vi "CC_T2_Manipulation.vi"(8 "Invert?":bool, 9 "Tau Step Size":dbl=2e-09, 10 "Numeric 2":i32, 11 "Numeric":i32) -> (2 "Tau":dbl)   [LabVIEW 2024]
uses:
  <vilib>/Utility/error.llb/DialogTypeEnum.ctl
  SpinCore_API_file_location.vi
panel:
  in  "# of Instructions":u32=33
  in  "Instructions":T1(array[cluster])=[{"Instruct Data"=0, "Op Code"=0, "Flags"=[FALSE, FALSE, TRUE, FALSE, FALSE, FALSE, FALSE, TRUE, FALSE, FALSE, FALSE, FALSE, FALSE, FALSE, FALSE, FALSE, FALSE, FALSE, FALSE, FALSE, FALSE, FALSE, FALSE, TRUE], "Comments"="0 Triggers", "Time (s)"=1e-07}, {"Instruct Data"=0, "Op Code"=0, "Flags"=[FALSE, FALSE, FALSE, FALSE, FALSE, FALSE, FALSE, TRUE, FALSE, FALSE, FALSE, FALSE, FALSE, FALSE, FALSE, FALSE, FALSE, FALSE, FALSE, FALSE, FALSE, FALSE, FALSE, FALSE], "Comments"="1 Dark ", "Time (s)"=5e-05}, {"Instruct Data"=0, "Op Code"=0, "Flags"=[FALSE, FALSE, FALSE, FALSE, FALSE, FALSE, FALSE, TRUE, FALSE, FALSE, FALSE, FALSE, FALSE, FALSE, FALSE, FALSE, FALSE, FALSE, FALSE, FALSE, FALSE, FALSE, FALSE, FALSE], "Comments"="2 AOM Buffer", "Time (s)"=5e-07}, {"Instruct Data"=0, "Op Code"=0, "Flags"=[TRUE, FALSE, FALSE, TRUE, FALSE, FALSE, FALSE, TRUE, FALSE, FALSE, FALSE, FALSE, FALSE, FALSE, FALSE, FALSE, FALSE, FALSE, FALSE, FALSE, FALSE, FALSE, FALSE, FALSE], "Comments"="3 pi/2_X", "Time (s)"=3.6e-08}, {"Instruct Data"=0, "Op Code"=0, "Flags"=[FALSE, FALSE, FALSE, FALSE, FALSE, FALSE, FALSE, TRUE, FALSE, FALSE, FALSE, FALSE, FALSE, FALSE, FALSE, FALSE, FALSE, FALSE, FALSE, FALSE, FALSE, FALSE, FALSE, FALSE], "Comments"="4 tau", "Time (s)"=2.1e-06}, {"Instruct Data"=0, "Op Code"=0, "Flags"=[TRUE, FALSE, FALSE, TRUE, FALSE, FALSE, FALSE, TRUE, FALSE, FALSE, FALSE, FALSE, FALSE, FALSE, FALSE, FALSE, FALSE, FALSE, FALSE, FALSE, FALSE, FALSE, FALSE, FALSE], "Comments"="5  Pi_X", "Time (s)"=6.7e-08}, {"Instruct Data"=0, "Op Code"=0, "Flags"=[FALSE, FALSE, FALSE, FALSE, FALSE, FALSE, FALSE, TRUE, FALSE, FALSE, FALSE, FALSE, FALSE, FALSE, FALSE, FALSE, FALSE, FALSE, FALSE, FALSE, FALSE, FALSE, FALSE, FALSE], "Comments"="6 Tau", "Time (s)"=2.1e-06}, {"Instruct Data"=0, "Op Code"=0, "Flags"=[TRUE, FALSE, FALSE, FALSE, TRUE, FALSE, FALSE, TRUE, FALSE, FALSE, FALSE, FALSE, FALSE, FALSE, FALSE, FALSE, FALSE, FALSE, FALSE, FALSE, FALSE, FALSE, FALSE, FALSE], "Comments"="7 Pi/2_Y", "Time (s)"=3.9e-08}, {"Instruct Data"=0, "Op Code"=0, "Flags"=[FALSE, FALSE, FALSE, FALSE, FALSE, FALSE, FALSE, TRUE, FALSE, FALSE, FALSE, FALSE, FALSE, FALSE, FALSE, FALSE, FALSE, FALSE, FALSE, FALSE, FALSE, FALSE, FALSE, FALSE], "Comments"="8 Tau CC", "Time (s)"=1e-08}, {"Instruct Data"=0, "Op Code"=0, "Flags"=[TRUE, FALSE, FALSE, TRUE, FALSE, FALSE, FALSE, TRUE, FALSE, FALSE, FALSE, FALSE, FALSE, FALSE, FALSE, FALSE, FALSE, FALSE, FALSE, FALSE, FALSE, FALSE, FALSE, FALSE], "Comments"="9 pi/2_X", "Time (s)"=3.6e-08}, {"Instruct Data"=0, "Op Code"=0, "Flags"=[FALSE, FALSE, FALSE, FALSE, FALSE, FALSE, FALSE, TRUE, FALSE, FALSE, FALSE, FALSE, FALSE, FALSE, FALSE, FALSE, FALSE, FALSE, FALSE, FALSE, FALSE, FALSE, FALSE, FALSE], "Comments"="10 tau", "Time (s)"=2.1e-06}, {"Instruct Data"=0, "Op Code"=0, "Flags"=[TRUE, FALSE, FALSE, TRUE, FALSE, FALSE, FALSE, TRUE, FALSE, FALSE, FALSE, FALSE, FALSE, FALSE, FALSE, FALSE, FALSE, FALSE, FALSE, FALSE, FALSE, FALSE, FALSE, FALSE], "Comments"="11  Pi_X", "Time (s)"=6.7e-08}, {"Instruct Data"=0, "Op Code"=0, "Flags"=[FALSE, FALSE, FALSE, FALSE, FALSE, FALSE, FALSE, TRUE, FALSE, FALSE, FALSE, FALSE, FALSE, FALSE, FALSE, FALSE, FALSE, FALSE, FALSE, FALSE, FALSE, FALSE, FALSE, FALSE], "Comments"="12 tau", "Time (s)"=2.1e-06}, {"Instruct Data"=0, "Op Code"=0, "Flags"=[TRUE, FALSE, FALSE, FALSE, TRUE, FALSE, FALSE, TRUE, FALSE, FALSE, FALSE, FALSE, FALSE, FALSE, FALSE, FALSE, FALSE, FALSE, FALSE, FALSE, FALSE, FALSE, FALSE, FALSE], "Comments"="13 pi/2_Y", "Time (s)"=3.7e-08}, {"Instruct Data"=0, "Op Code"=0, "Flags"=[FALSE, TRUE, FALSE, FALSE, FALSE, FALSE, FALSE, TRUE, FALSE, FALSE, FALSE, FALSE, FALSE, FALSE, FALSE, FALSE, FALSE, FALSE, FALSE, FALSE, FALSE, FALSE, FALSE, FALSE], "Comments"="14 AOM Delay", "Time (s)"=5e-07}, {"Instruct Data"=0, "Op Code"=0, "Flags"=[FALSE, TRUE, FALSE, FALSE, FALSE, FALSE, FALSE, FALSE, FALSE, FALSE, FALSE, FALSE, FALSE, FALSE, FALSE, FALSE, FALSE, FALSE, FALSE, FALSE, FALSE, FALSE, FALSE, FALSE], "Comments"="15 inhibit off", "Time (s)"=5e-07}, {"Instruct Data"=0, "Op Code"=0, "Flags"=[FALSE, TRUE, FALSE, FALSE, FALSE, FALSE, FALSE, TRUE, FALSE, FALSE, FALSE, FALSE, FALSE, FALSE, FALSE, FALSE, FALSE, FALSE, FALSE, FALSE, FALSE, FALSE, FALSE, FALSE], "Comments"="16 AOM", "Time (s)"=5e-06}, {"Instruct Data"=0, "Op Code"=0, "Flags"=[FALSE, FALSE, FALSE, FALSE, FALSE, FALSE, FALSE, TRUE, FALSE, FALSE, FALSE, FALSE, FALSE, FALSE, FALSE, FALSE, FALSE, FALSE, FALSE, FALSE, FALSE, FALSE, FALSE, FALSE], "Comments"="17 Dark", "Time (s)"=5e-05}, {"Instruct Data"=0, "Op Code"=0, "Flags"=[FALSE, FALSE, FALSE, FALSE, FALSE, FALSE, FALSE, TRUE, FALSE, FALSE, FALSE, FALSE, FALSE, FALSE, FALSE, FALSE, FALSE, FALSE, FALSE, FALSE, FALSE, FALSE, FALSE, FALSE], "Comments"="18 AOM Delay", "Time (s)"=5e-07}, {"Instruct Data"=0, "Op Code"=0, "Flags"=[TRUE, FALSE, FALSE, TRUE, FALSE, FALSE, FALSE, TRUE, FALSE, FALSE, FALSE, FALSE, FALSE, FALSE, FALSE, FALSE, FALSE, FALSE, FALSE, FALSE, FALSE, FALSE, FALSE, FALSE], "Comments"="19 pi/2_X ", "Time (s)"=3.6e-08}, {"Instruct Data"=0, "Op Code"=0, "Flags"=[FALSE, FALSE, FALSE, FALSE, FALSE, FALSE, FALSE, TRUE, FALSE, FALSE, FALSE, FALSE, FALSE, FALSE, FALSE, FALSE, FALSE, FALSE, FALSE, FALSE, FALSE, FALSE, FALSE, FALSE], "Comments"="20 tau", "Time (s)"=2.1e-06}, {"Instruct Data"=0, "Op Code"=0, "Flags"=[TRUE, FALSE, FALSE, TRUE, FALSE, FALSE, FALSE, TRUE, FALSE, FALSE, FALSE, FALSE, FALSE, FALSE, FALSE, FALSE, FALSE, FALSE, FALSE, FALSE, FALSE, FALSE, FALSE, FALSE], "Comments"="21 Pi_x", "Time (s)"=6.7e-08}, {"Instruct Data"=0, "Op Code"=0, "Flags"=[FALSE, FALSE, FALSE, FALSE, FALSE, FALSE, FALSE, TRUE, FALSE, FALSE, FALSE, FALSE, FALSE, FALSE, FALSE, FALSE, FALSE, FALSE, FALSE, FALSE, FALSE, FALSE, FALSE, FALSE], "Comments"="22 tau", "Time (s)"=2.1e-06}, {"Instruct Data"=0, "Op Code"=0, "Flags"=[TRUE, FALSE, FALSE, FALSE, TRUE, FALSE, FALSE, TRUE, FALSE, FALSE, FALSE, FALSE, FALSE, FALSE, FALSE, FALSE, FALSE, FALSE, FALSE, FALSE, FALSE, FALSE, FALSE, FALSE], "Comments"="23 pi/2 _Y", "Time (s)"=3.9e-08}, {"Instruct Data"=0, "Op Code"=0, "Flags"=[FALSE, FALSE, FALSE, FALSE, FALSE, FALSE, FALSE, TRUE, FALSE, FALSE, FALSE, FALSE, FALSE, FALSE, FALSE, FALSE, FALSE, FALSE, FALSE, FALSE, FALSE, FALSE, FALSE, FALSE], "Comments"="24 Tau_CC", "Time (s)"=1e-08}, {"Instruct Data"=0, "Op Code"=0, "Flags"=[TRUE, FALSE, FALSE, TRUE, FALSE, FALSE, FALSE, TRUE, FALSE, FALSE, FALSE, FALSE, FALSE, FALSE, FALSE, FALSE, FALSE, FALSE, FALSE, FALSE, FALSE, FALSE, FALSE, FALSE], "Comments"="25 pi/2_X", "Time (s)"=3.6e-08}, {"Instruct Data"=0, "Op Code"=0, "Flags"=[FALSE, FALSE, FALSE, FALSE, FALSE, FALSE, FALSE, TRUE, FALSE, FALSE, FALSE, FALSE, FALSE, FALSE, FALSE, FALSE, FALSE, FALSE, FALSE, FALSE, FALSE, FALSE, FALSE, FALSE], "Comments"="26 tau", "Time (s)"=2.1e-06}, {"Instruct Data"=0, "Op Code"=0, "Flags"=[TRUE, FALSE, FALSE, TRUE, FALSE, FALSE, FALSE, TRUE, FALSE, FALSE, FALSE, FALSE, FALSE, FALSE, FALSE, FALSE, FALSE, FALSE, FALSE, FALSE, FALSE, FALSE, FALSE, FALSE], "Comments"="27 Pi_X", "Time (s)"=6.7e-08}, {"Instruct Data"=0, "Op Code"=0, "Flags"=[FALSE, FALSE, FALSE, FALSE, FALSE, FALSE, FALSE, TRUE, FALSE, FALSE, FALSE, FALSE, FALSE, FALSE, FALSE, FALSE, FALSE, FALSE, FALSE, FALSE, FALSE, FALSE, FALSE, FALSE], "Comments"="28 tau", "Time (s)"=2.1e-06}, {"Instruct Data"=0, "Op Code"=0, "Flags"=[TRUE, FALSE, FALSE, FALSE, TRUE, FALSE, FALSE, TRUE, FALSE, FALSE, FALSE, FALSE, FALSE, FALSE, FALSE, FALSE, FALSE, FALSE, FALSE, FALSE, FALSE, FALSE, FALSE, FALSE], "Comments"="29 3pi/2_Y", "Time (s)"=1.05e-07}, {"Instruct Data"=0, "Op Code"=0, "Flags"=[FALSE, TRUE, FALSE, FALSE, FALSE, FALSE, FALSE, TRUE, FALSE, FALSE, FALSE, FALSE, FALSE, FALSE, FALSE, FALSE, FALSE, FALSE, FALSE, FALSE, FALSE, FALSE, FALSE, FALSE], "Comments"="30  aom delay", "Time (s)"=5e-07}, {"Instruct Data"=0, "Op Code"=0, "Flags"=[FALSE, TRUE, FALSE, FALSE, FALSE, FALSE, FALSE, FALSE, FALSE, FALSE, FALSE, FALSE, FALSE, FALSE, FALSE, FALSE, FALSE, FALSE, FALSE, FALSE, FALSE, FALSE, FALSE, FALSE], "Comments"="31inhibit off", "Time (s)"=5e-07}, {"Instruct Data"=0, "Op Code"=6, "Flags"=[FALSE, TRUE, FALSE, FALSE, FALSE, FALSE, FALSE, TRUE, FALSE, FALSE, FALSE, FALSE, FALSE, FALSE, FALSE, FALSE, FALSE, FALSE, FALSE, FALSE, FALSE, FALSE, FALSE, FALSE], "Comments"="32  aom", "Time (s)"=5e-06}, {"Instruct Data"=0, "Op Code"=0, "Flags"=[TRUE, FALSE, FALSE, TRUE, FALSE, FALSE, FALSE, TRUE, FALSE, FALSE, FALSE, FALSE, FALSE, FALSE, FALSE, FALSE, FALSE, FALSE, FALSE, FALSE, FALSE, FALSE, FALSE, FALSE], "Comments"="33 AOM", "Time (s)"=9.2e-08}] {"Time (s)" format="%.3p"; "Op Code" items=["Continue", "Stop", "Loop", "End Loop", "JSR", "RTS", "Branch", "Long Delay", "Wait"]}
  out "output array":T1(array[cluster])
  in  "clock_freq (MHz)":dbl=500.0
  out "x+y 2":dbl
  out "x+y 5":dbl
  out "x+y 6":dbl
  out "output array 2":T1(array[cluster])
  in  "clock_freq (MHz) 2":dbl=500.0
  out "x+y 11":dbl
  out "x+y 8":dbl
  out "x+y 7":dbl
  # "1) MW indication\n2)AOM\n3) SR400 trigger\n4) I\n5) Q\n8) inhibit\n24) oss trigger"
  # "1"
  # "2"
  # "3"
  # "4"
  # "5"
  # "6"
  # "7"
  # "8"
  # "9"
  # "10"
  # "11"
  # "12"
  # "13"
  # "14"
  # "15"
  # "16"
  # "17"
  # "18"
  # "19"
  # "20"
  # "21"
  # "22"
  # "23"
  # "24"
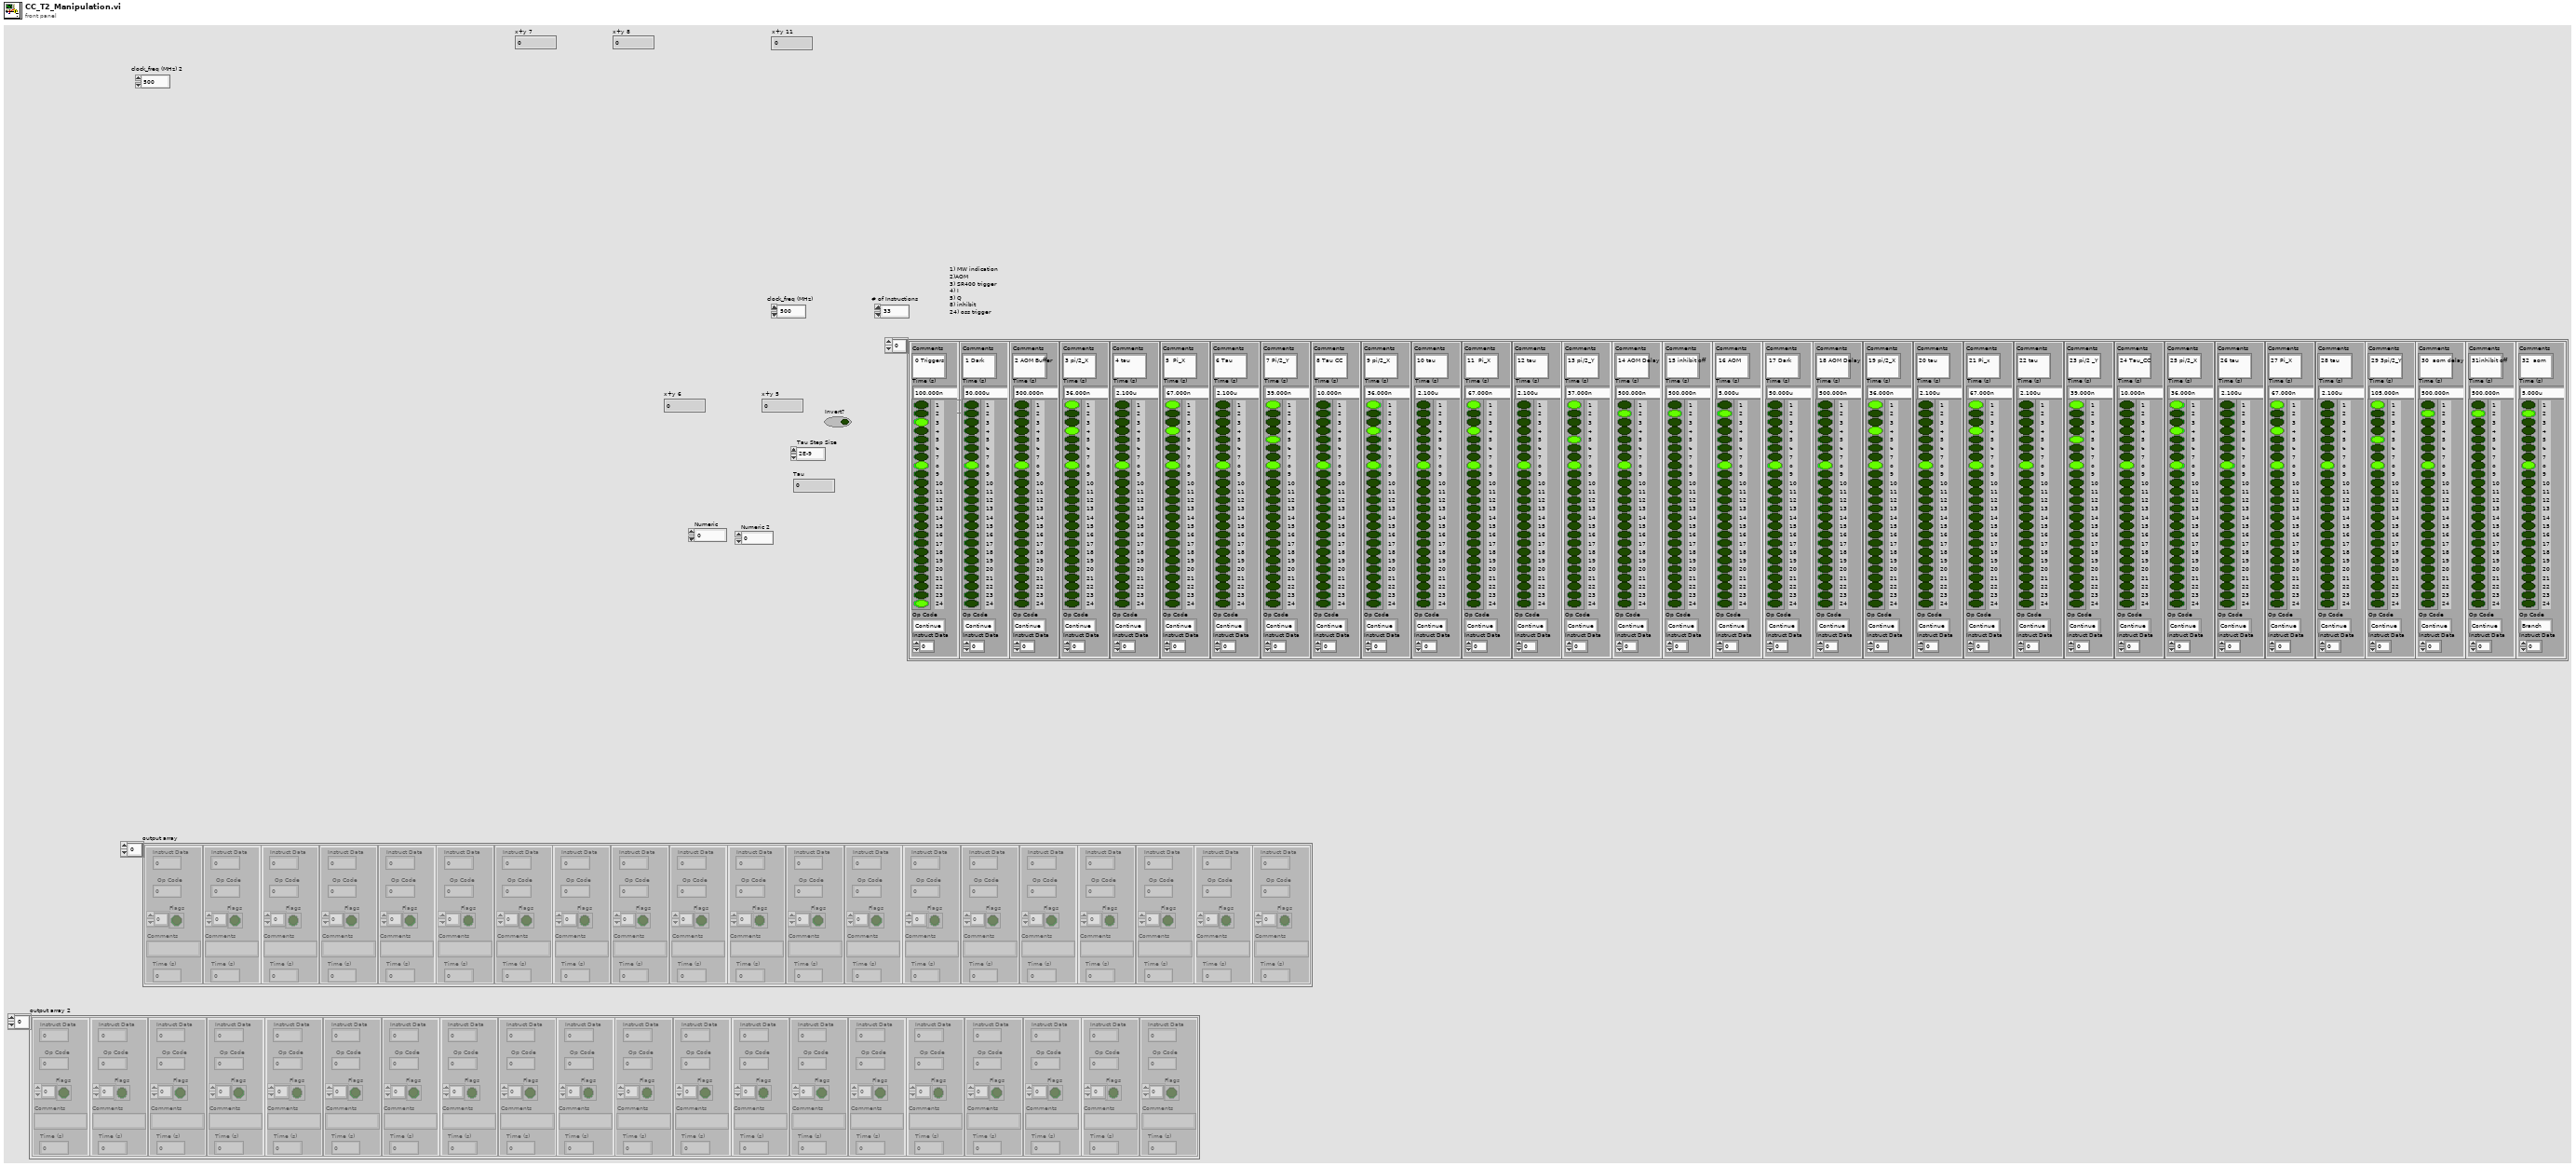
[diagram p1: front panel]
types:
  T1 = cluster{"Instruct Data":i32, "Op Code":i32, "Flags":bool[], "Comments":string, "Time (s)":dbl}[]
  T2 = typedef "DialogTypeEnum.ctl" = enum16{"no dialog", "OK message", "continue or stop message", "auto error handling dialog", "OK message + warnings", "continue/stop + warnings"}
  T3 = enum16{"Pulse Program", "Frequency Registers", "TX Phase Registers", "RX Phase Registers"}
  T4 = cluster{"Instruct Data":i32, "Op Code":i32, "Flags":bool[], "Comments":string, "Time (s)":dbl}
  T5 = cluster{"Instruct Data":i32, "Op Code":i32, "Flags":bool[], "Comments":string, dbl}
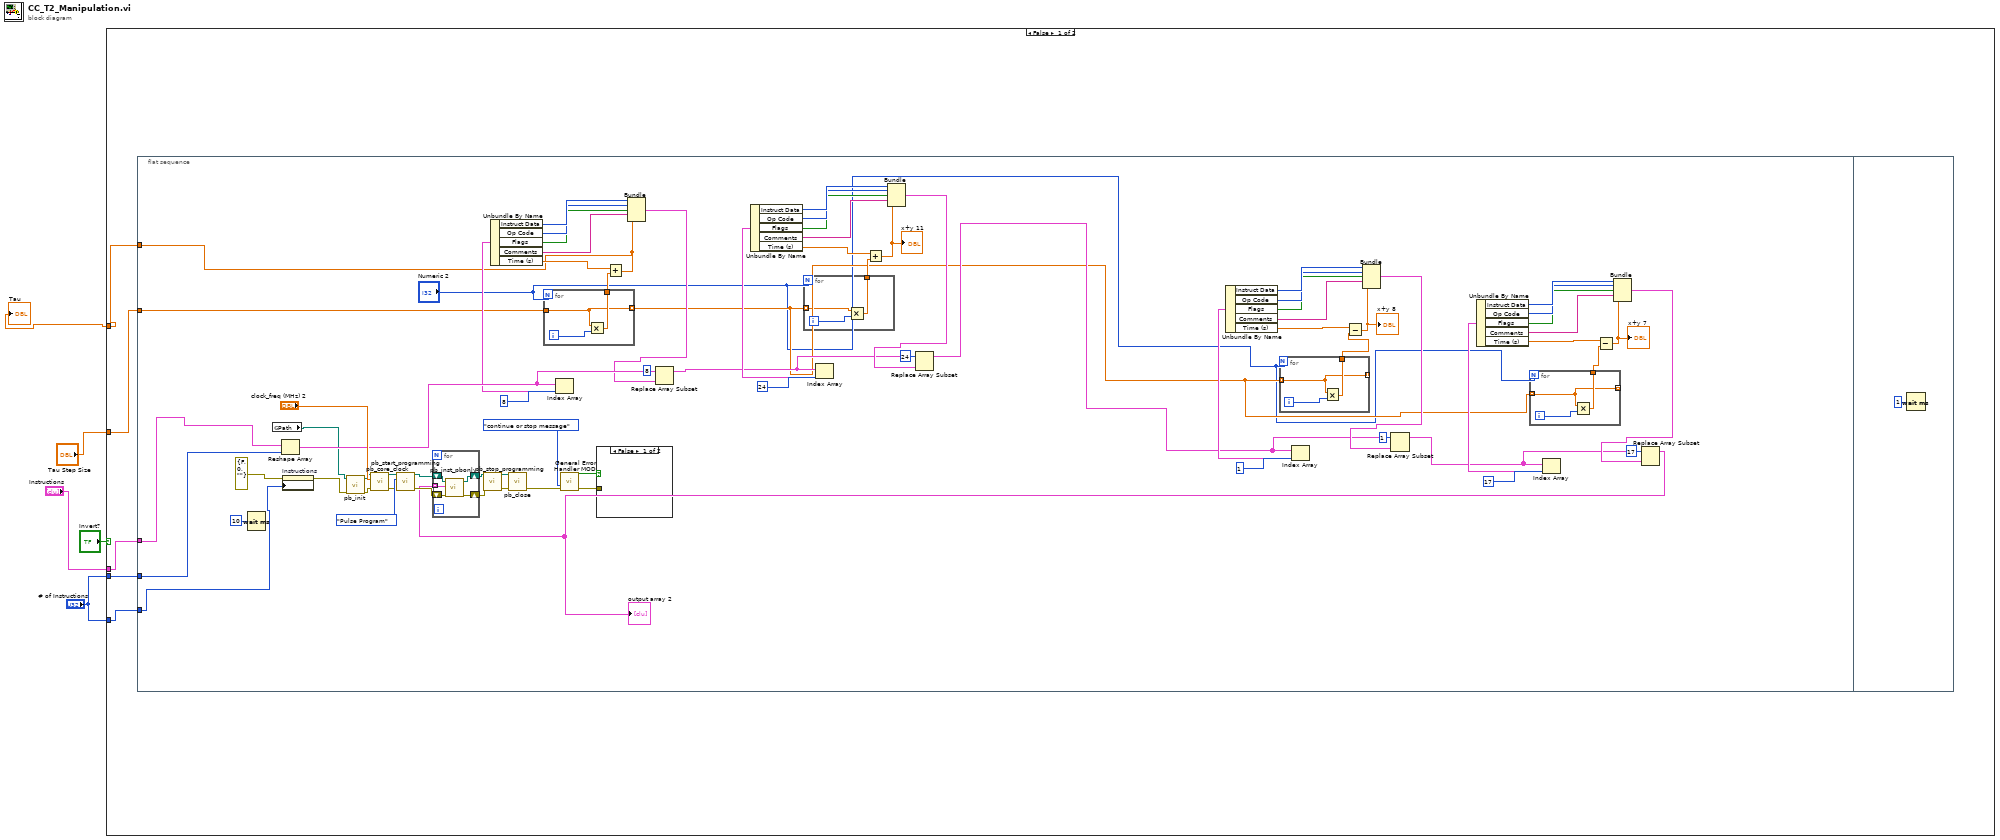
[diagram p0: block diagram]
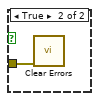
[diagram p2: hidden frame]
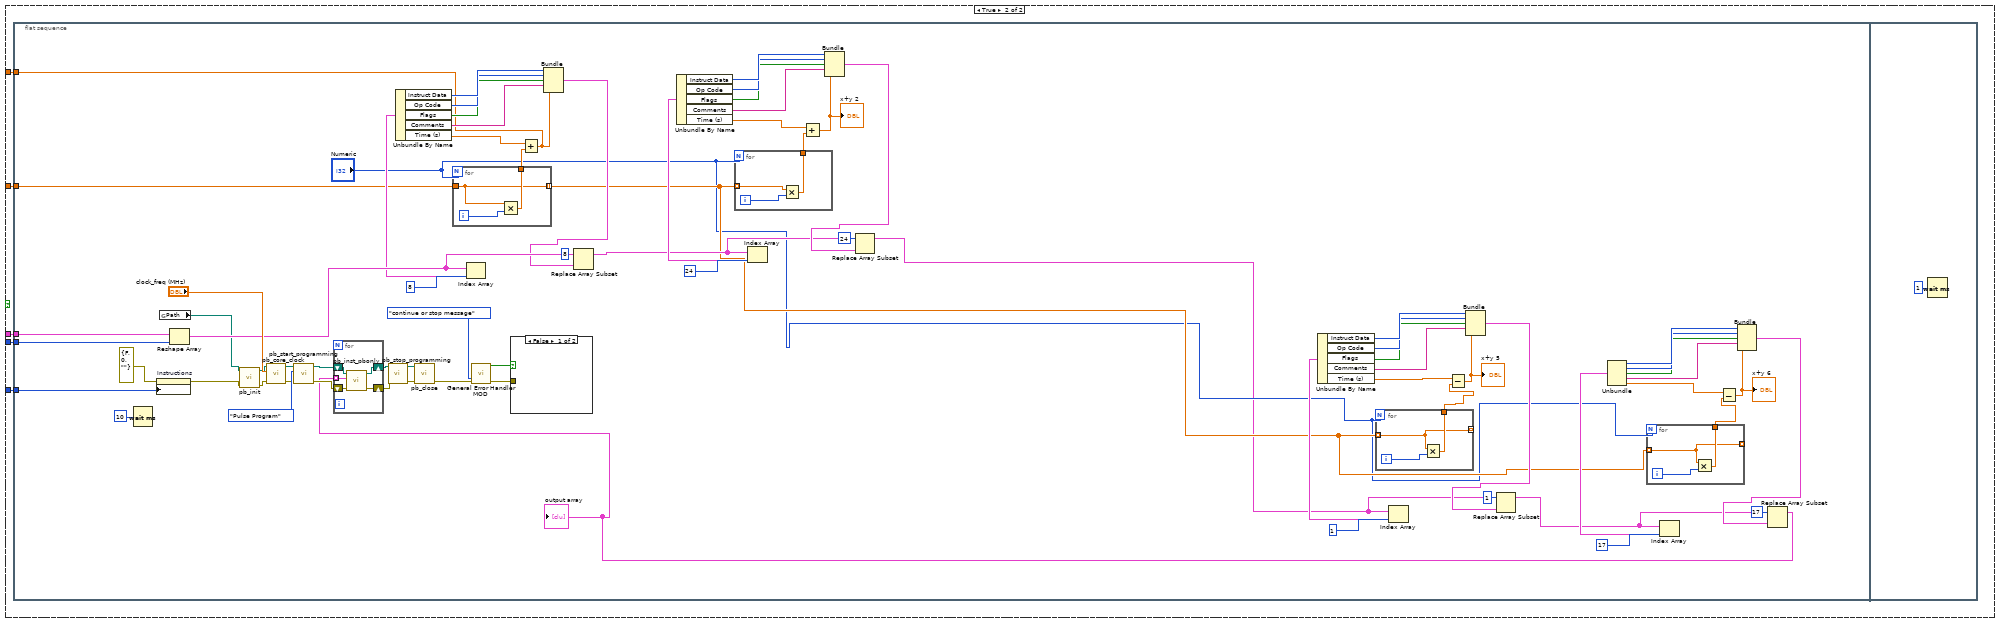
[diagram p3: hidden frame]
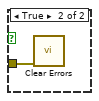
[diagram p4: hidden frame]
diagram:
  n1 = case shown="False" "Invert?" {
    tunnel: "Instructions" -> [w10 w109]
    tunnel: "# of Instructions" -> [w9 w108]
    tunnel: "# of Instructions" -> [w8 w107]
    tunnel: "Tau Step Size" -> [w7 w106]
    tunnel: [w6 w105] -> w1
    frame False {
      n2 = flat-sequence {
        tunnel: w10 -> [w23]
        tunnel: w9 -> [w22]
        tunnel: w8 -> [w21]
        tunnel: w7 -> [w17]
        tunnel: [w16] -> w6
        frame #0 {
          n3 = Wait (ms)(milliseconds to wait=u32 10) -> ()  [unwired: 1 out]
          n4 = global read "SpinCore_API_file_location.vi" "Path"() -> (w18:path)
          n5 = Reshape Array "Reshape Array"(w23, w22) -> (w65:T1)
          n6 = property on="Instructions" class="Arr (strict)"(error in=errorcluster {"status"=FALSE, "code"=0, "source"=""} ("error in (no error)"), "Number of Columns"=w21) -> (error out=w19:errorcluster)  [unwired: 1 in, 1 out]
          n7 = call "pb_init.vi"("error in (no error)"=w19, "path in"=w18) -> ("error out"=w60:errorcluster, "path out"=w59:path)  [unwired: 8 in]
          n8 = call "pb_core_clock.vi"("error in (no error)"=w60, "clock_freq (MHz)"="clock_freq (MHz) 2", "path in"=w59) -> ("error out"=w74:errorcluster, "path out"=w75:path)  [unwired: 7 in]
          n9 = call "pb_start_programming.vi"("error in (no error)"=w74, "Device"=T3."Pulse Program", "path in"=w75) -> ("error out"=w81:errorcluster, "path out"=w85:path)  [unwired: 1 in, 6 out]
          n10 = for {
            N: "Numeric 2" -> [_]
            tunnel: [w96] -> w61
            tunnel: [w95] -> w12 mode=indexing
            tunnel: w17 -> [w95]
            i -> [w97]
            n11 = Multiply(x=w95, y=w97) -> (x*y=w96:dbl)
          }
          n12 = Index Array "Index Array"(array=w65, index=8) -> (element=w64:T4)
          n13 = Unbundle By Name "Unbundle By Name"(w64) -> ("Instruct Data"=w70:i32, "Op Code"=w69:i32, "Flags"=w68:bool[], "Comments"=w67:string, "Time (s)"=w66:dbl)
          n14 = Add(x=w66, y=w61) -> (x+y=w16:dbl)
          n15 = Bundle("Instruct Data"=w70, "Op Code"=w69, "Flags"=w68, "Comments"=w67, w16) -> (w62:T5)  [unwired: 1 in]
          n16 = Replace Array Subset "Replace Array Subset"(array=w65, new element=w62, index=8) -> (w46:T1)
          n17 = for {
            N: "Numeric 2" -> [_]
            tunnel: [w93] -> w47
            tunnel: w12 -> [w92] mode=indexing
            i -> [w94]
            n18 = Multiply(x=w92, y=w94) -> (x*y=w93:dbl)
          }
          n19 = Index Array "Index Array"(array=w46, index=24) -> (element=w50:T4)
          n20 = Unbundle By Name "Unbundle By Name"(w50) -> ("Instruct Data"=w56:i32, "Op Code"=w55:i32, "Flags"=w54:bool[], "Comments"=w53:string, "Time (s)"=w52:dbl)
          n21 = Add(x=w52, y=w47) -> (x+y=w51:dbl)
          "x+y 11" <- w51
          n22 = Bundle("Instruct Data"=w56, "Op Code"=w55, "Flags"=w54, "Comments"=w53, w51) -> (w48:T5)  [unwired: 1 in]
          n23 = Replace Array Subset "Replace Array Subset"(array=w46, new element=w48, index=24) -> (w13:T1)
          n24 = for {
            N: "Numeric 2" -> [_]
            tunnel: [w90] -> w15
            tunnel: [w89] -> _ mode=indexing
            tunnel: w12 -> [w89] mode=indexing
            i -> [w91]
            n25 = Multiply(x=w89, y=w91) -> (x*y=w90:dbl)
          }
          n26 = Index Array "Index Array"(array=w13, index=1) -> (element=w38:T4)
          n27 = Unbundle By Name "Unbundle By Name"(w38) -> ("Instruct Data"=w44:i32, "Op Code"=w43:i32, "Flags"=w42:bool[], "Comments"=w41:string, "Time (s)"=w40:dbl)
          n28 = Subtract(x=w40, y=w15) -> (x-y=w39:dbl)
          "x+y 8" <- w39
          n29 = Bundle("Instruct Data"=w44, "Op Code"=w43, "Flags"=w42, "Comments"=w41, w39) -> (w36:T5)  [unwired: 1 in]
          n30 = Replace Array Subset "Replace Array Subset"(array=w13, new element=w36, index=1) -> (w25:T1)
          n31 = for {
            N: "Numeric 2" -> [_]
            tunnel: [w87] -> w14
            tunnel: [w86] -> _ mode=indexing
            tunnel: w12 -> [w86] mode=indexing
            i -> [w88]
            n32 = Multiply(x=w86, y=w88) -> (x*y=w87:dbl)
          }
          n33 = Index Array "Index Array"(array=w25, index=17) -> (element=w28:T4)
          n34 = Unbundle By Name "Unbundle By Name"(w28) -> ("Instruct Data"=w34:i32, "Op Code"=w33:i32, "Flags"=w32:bool[], "Comments"=w31:string, "Time (s)"=w30:dbl)
          n35 = Subtract(x=w30, y=w14) -> (x-y=w29:dbl)
          "x+y 7" <- w29
          n36 = Bundle("Instruct Data"=w34, "Op Code"=w33, "Flags"=w32, "Comments"=w31, w29) -> (w26:T5)  [unwired: 1 in]
          n37 = Replace Array Subset "Replace Array Subset"(array=w25, new element=w26, index=17) -> (w24:T1)
          "output array 2" <- w24
          n38 = for {
            tunnel: w24 -> [w100] mode=indexing
            shift-right: [w102] -> w83
            shift-left: w85 -> [w103]
            shift-right: [w99] -> w80
            shift-left: w81 -> [w101]
            n39 = call "pb_inst_pbonly.vi"("error in (no error)"=w101, "PB Instruction"=w100, "path in"=w103) -> ("error out"=w99:errorcluster, "path out"=w102:path)  [unwired: 2 in, 5 out]
          }
          n40 = call "pb_stop_programming.vi"("error in (no error)"=w80, "path in"=w83) -> ("error out"=w79:errorcluster, "path out"=w84:path)  [unwired: 1 in, 7 out]
          n41 = call "pb_close.vi"("error in (no error)"=w79, "path in"=w84) -> ("error out"=w72:errorcluster)  [unwired: 9 out]
          n42 = call "General Error Handler MOD.vi"("type of dialog (OK msg:1)"=DialogTypeEnum."continue or stop message", "error in (no error)"=w72) -> ("STOP?"=w76:bool, "error out"=w77:errorcluster)  [unwired: 12 out]
          n43 = case shown="False" w76 {
            tunnel: w77 -> [_ w98]
            frame False {
            }
            frame True {
              n44 = call <vilib>:"Clear Errors.vi"("error in (no error)"=w98) -> ()  [unwired: 1 in, 6 out]
            }
          }
        }
        frame #1 {
          n45 = Wait (ms)(milliseconds to wait=u32 1) -> ()  [unwired: 1 out]
        }
      }
    }
    frame True {
      n46 = flat-sequence {
        tunnel: w109 -> [w119]
        tunnel: w108 -> [w118]
        tunnel: w107 -> [w117]
        tunnel: w106 -> [w116]
        tunnel: [w115] -> w105
        frame #0 {
          n47 = Wait (ms)(milliseconds to wait=u32 10) -> ()  [unwired: 1 out]
          n48 = property on="Instructions" class="Arr (strict)"(error in=errorcluster {"status"=FALSE, "code"=0, "source"=""} ("error in (no error)"), "Number of Columns"=w117) -> (error out=w158:errorcluster)  [unwired: 1 in, 1 out]
          n49 = global read "SpinCore_API_file_location.vi" "Path"() -> (w159:path)
          n50 = Reshape Array "Reshape Array"(w119, w118) -> (w164:T1)
          n51 = call "pb_init.vi"("error in (no error)"=w158, "path in"=w159) -> ("error out"=w157:errorcluster, "path out"=w156:path)  [unwired: 8 in]
          n52 = call "pb_core_clock.vi"("error in (no error)"=w157, "clock_freq (MHz)"="clock_freq (MHz)", "path in"=w156) -> ("error out"=w173:errorcluster, "path out"=w174:path)  [unwired: 7 in]
          n53 = call "pb_start_programming.vi"("error in (no error)"=w173, "Device"=T3."Pulse Program", "path in"=w174) -> ("error out"=w180:errorcluster, "path out"=w184:path)  [unwired: 1 in, 6 out]
          n54 = for {
            N: "Numeric" -> [_]
            tunnel: [w195] -> w160
            tunnel: [w194] -> w114 mode=indexing
            tunnel: w116 -> [w194]
            i -> [w196]
            n55 = Multiply(x=w194, y=w196) -> (x*y=w195:dbl)
          }
          n56 = Index Array "Index Array"(array=w164, index=8) -> (element=w163:T4)
          n57 = Unbundle By Name "Unbundle By Name"(w163) -> ("Instruct Data"=w169:i32, "Op Code"=w168:i32, "Flags"=w167:bool[], "Comments"=w166:string, "Time (s)"=w165:dbl)
          n58 = Add(x=w165, y=w160) -> (x+y=w115:dbl)
          n59 = Bundle("Instruct Data"=w169, "Op Code"=w168, "Flags"=w167, "Comments"=w166, w115) -> (w161:T5)  [unwired: 1 in]
          n60 = Replace Array Subset "Replace Array Subset"(array=w164, new element=w161, index=8) -> (w142:T1)
          n61 = for {
            N: "Numeric" -> [_]
            tunnel: [w192] -> w143
            tunnel: w114 -> [w191] mode=indexing
            i -> [w193]
            n62 = Multiply(x=w191, y=w193) -> (x*y=w192:dbl)
          }
          n63 = Index Array "Index Array"(array=w142, index=24) -> (element=w146:T4)
          n64 = Unbundle By Name "Unbundle By Name"(w146) -> ("Instruct Data"=w152:i32, "Op Code"=w151:i32, "Flags"=w150:bool[], "Comments"=w149:string, "Time (s)"=w148:dbl)
          n65 = Add(x=w148, y=w143) -> (x+y=w147:dbl)
          "x+y 2" <- w147
          n66 = Bundle("Instruct Data"=w152, "Op Code"=w151, "Flags"=w150, "Comments"=w149, w147) -> (w144:T5)  [unwired: 1 in]
          n67 = Replace Array Subset "Replace Array Subset"(array=w142, new element=w144, index=24) -> (w112:T1)
          n68 = for {
            N: "Numeric" -> [_]
            tunnel: [w189] -> w111
            tunnel: [w188] -> _ mode=indexing
            tunnel: w114 -> [w188] mode=indexing
            i -> [w190]
            n69 = Multiply(x=w188, y=w190) -> (x*y=w189:dbl)
          }
          n70 = Index Array "Index Array"(array=w112, index=1) -> (element=w134:T4)
          n71 = Unbundle By Name "Unbundle By Name"(w134) -> ("Instruct Data"=w140:i32, "Op Code"=w139:i32, "Flags"=w138:bool[], "Comments"=w137:string, "Time (s)"=w136:dbl)
          n72 = Subtract(x=w136, y=w111) -> (x-y=w135:dbl)
          "x+y 5" <- w135
          n73 = Bundle("Instruct Data"=w140, "Op Code"=w139, "Flags"=w138, "Comments"=w137, w135) -> (w132:T5)  [unwired: 1 in]
          n74 = Replace Array Subset "Replace Array Subset"(array=w112, new element=w132, index=1) -> (w121:T1)
          n75 = for {
            N: "Numeric" -> [_]
            tunnel: [w186] -> w110
            tunnel: [w185] -> _ mode=indexing
            tunnel: w114 -> [w185] mode=indexing
            i -> [w187]
            n76 = Multiply(x=w185, y=w187) -> (x*y=w186:dbl)
          }
          n77 = Index Array "Index Array"(array=w121, index=17) -> (element=w124:T4)
          n78 = Unbundle(w124) -> ("Instruct Data"=w130:i32, "Op Code"=w129:i32, "Flags"=w128:bool[], "Comments"=w127:string, "Time (s)"=w126:dbl)
          n79 = Subtract(x=w126, y=w110) -> (x-y=w125:dbl)
          "x+y 6" <- w125
          n80 = Bundle("Instruct Data"=w130, "Op Code"=w129, "Flags"=w128, "Comments"=w127, w125) -> (w122:T5)  [unwired: 1 in]
          n81 = Replace Array Subset "Replace Array Subset"(array=w121, new element=w122, index=17) -> (w120:T1)
          "output array" <- w120
          n82 = for {
            tunnel: w120 -> [w199] mode=indexing
            shift-right: [w201] -> w182
            shift-left: w184 -> [w202]
            shift-right: [w198] -> w179
            shift-left: w180 -> [w200]
            n83 = call "pb_inst_pbonly.vi"("error in (no error)"=w200, "PB Instruction"=w199, "path in"=w202) -> ("error out"=w198:errorcluster, "path out"=w201:path)  [unwired: 2 in, 5 out]
          }
          n84 = call "pb_stop_programming.vi"("error in (no error)"=w179, "path in"=w182) -> ("error out"=w178:errorcluster, "path out"=w183:path)  [unwired: 1 in, 7 out]
          n85 = call "pb_close.vi"("error in (no error)"=w178, "path in"=w183) -> ("error out"=w171:errorcluster)  [unwired: 9 out]
          n86 = call "General Error Handler MOD.vi"("type of dialog (OK msg:1)"=DialogTypeEnum."continue or stop message", "error in (no error)"=w171) -> ("STOP?"=w175:bool, "error out"=w176:errorcluster)  [unwired: 12 out]
          n87 = case shown="False" w175 {
            tunnel: w176 -> [_ w197]
            frame False {
            }
            frame True {
              n88 = call <vilib>:"Clear Errors.vi"("error in (no error)"=w197) -> ()  [unwired: 1 in, 6 out]
            }
          }
        }
        frame #1 {
          n89 = Wait (ms)(milliseconds to wait=u32 1) -> ()  [unwired: 1 out]
        }
      }
    }
  }
  "Tau" <- w1
